vi "Find Tests.vi"(8 "error in (no error)":errorcluster, 10 "Project Refnum":refnum<vi>, 11 "LVUnit Test Discoverer in":refnum<class "LVUnit Test Discoverer.lvclass">) -> (0 "error out":errorcluster, 2 "Test Cases":refnum<class "Test Case.lvclass">[](array[class]), 3 "LVUnit Test Discoverer out":refnum<class "LVUnit Test Discoverer.lvclass">)   [LabVIEW 2017, in "LVUnit Test Discoverer.lvclass"]
doc: "Finds the tests available from the specified project refnum."
uses:
  LVUnit Test Discoverer.lvclass
  Test Case/Test Case.lvclass
  LVUnit Test Case/LVUnit Test Case.lvclass
  C:/Users/pasca/source/repos/lvunit/Test Case/Test Case.lvclass
  LVUnit Test Case/LVUnit Test Case.lvclass/LVUnit Test Case.ctl
  2d6a42ca-fa2d-47c0-93bd-f8bf5f61b6df.vi
  LVUnit Test Case/Set JSON Data.vi
  <vilib>/JDP Science/JSONtext/JSON text to Variant.vi
  <vilib>/JDP Science/JSONtext/LVClass Serializer/JSONtext LVClass Serializer.lvclass
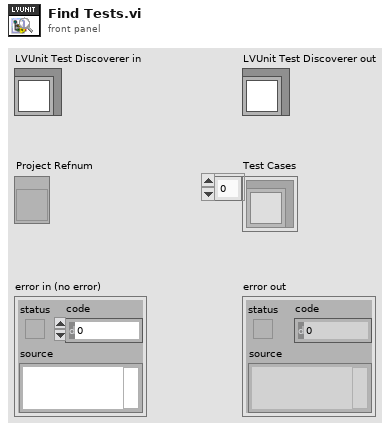
[diagram p1: front panel]
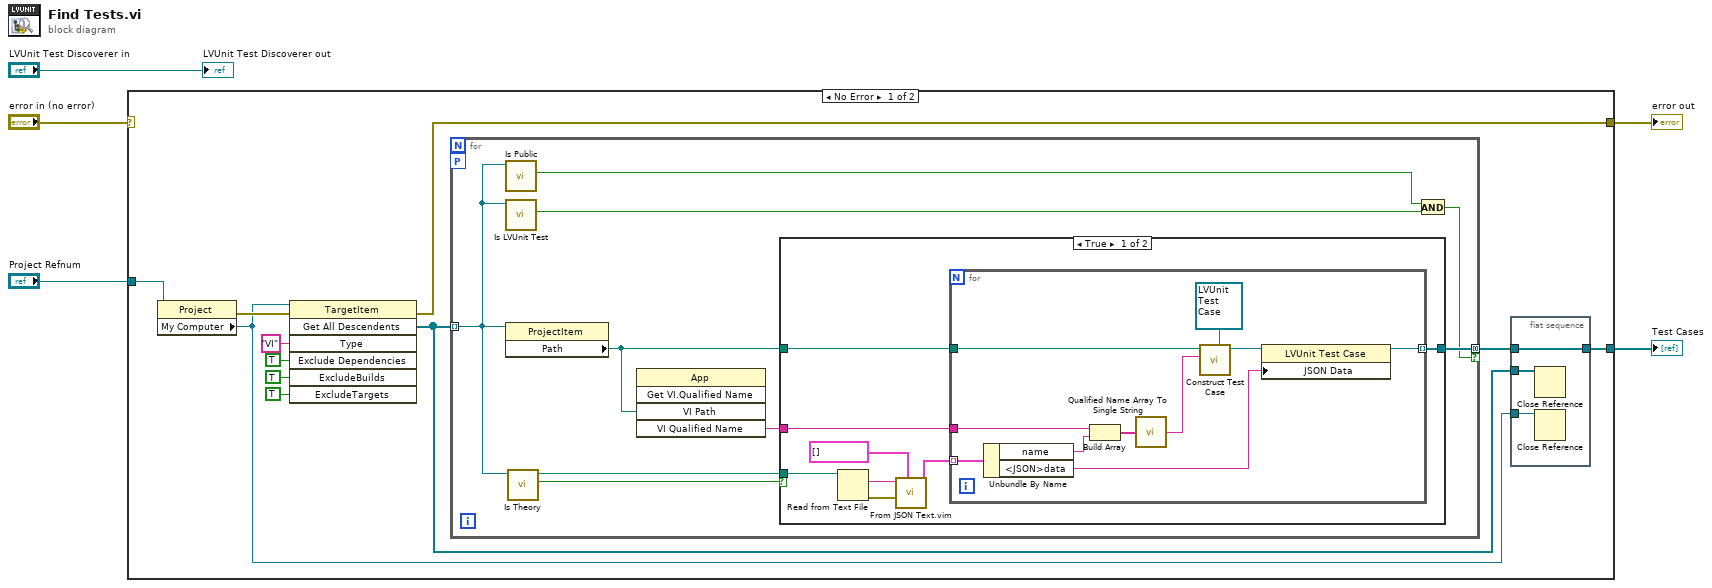
[diagram p0: block diagram]
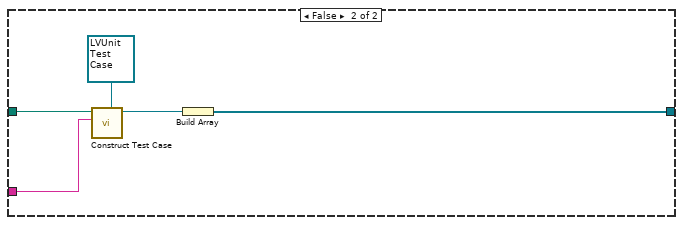
[diagram p2: hidden frame]
diagram:
  n1 = case shown="No Error" "error in (no error)" {
    selector: "error in (no error)" -> [_ w52]
    tunnel: "Project Refnum" -> [w16 _]
    tunnel: [w9 _] -> w3
    tunnel: [w12 w52] -> w2
    frame No Error {
      n2 = property class="Project"(reference=w16) -> (error out=w13:errorcluster, "My Computer"=w6:refnum<vi>)  [unwired: 1 in, 1 out]
      n3 = invoke class="TargetItem" method="Get All Descendents"(reference=w6, error in=w13, "Type"="VI", "Exclude Dependencies"=TRUE ("ExcludeDependencies"), "ExcludeBuilds"=TRUE, "ExcludeTargets"=TRUE) -> (error out=w12:errorcluster, "All Descendents"=w7:refnum<vi>[])  [unwired: 1 in, 5 out]
      n4 = for {
        tunnel: w7 -> [w25] mode=indexing
        tunnel: [w28] -> w8 mode=concatenating if=w22
        workers-P: _ -> [_]
        n5 = call "Is Public.vi"("ProjectItem Refnum"=w25) -> ("Is Public"=w23:bool)  [unwired: 10 in]
        n6 = call "Is LVUnit Test.vi"("ProjectItem Refnum"=w25) -> ("Is LVUnit Test"=w24:bool)  [unwired: 10 in]
        n7 = property class="ProjectItem"(reference=w25) -> ("Path"=w21:path)  [unwired: 1 in, 2 out]
        n8 = call "Is Theory.vi"("ProjectItem Refnum"=w25) -> ("Is Theory"=w26:bool, "Json File"=w27:path)  [unwired: 9 in]
        n9 = invoke class="App" method="Get VI.Qualified Name"("VI Path"=w21) -> ("VI Qualified Name"=w20:string)  [unwired: 4 in, 4 out]
        n10 = case shown="True" w26 {
          tunnel: [w36 w49] -> w28
          tunnel: w21 -> [w35 w50]
          tunnel: w27 -> [w30 _]
          tunnel: w20 -> [w34 w48]
          frame True {
            n11 = Read from Text File(file (use dialog)=w30) -> (text=w33:string, error out=w32:errorcluster)  [unwired: 3 in, 2 out]
            n12 = call "From JSON Text.vim"("Data Type and Default Value"=cluster{"name":string, "<JSON>data":string}[] [], "error in (no error)"=w32, "JSON"=w33) -> ("Data out"=w29:cluster{"name":string, "<JSON>data":string}[])  [unwired: 7 in, 1 out]
            n13 = for {
              tunnel: [w40] -> w36 mode=indexing
              tunnel: w35 -> [w45]
              tunnel: w34 -> [w44]
              tunnel: w29 -> [w39] mode=indexing
              n14 = Unbundle By Name(w39) -> ("name"=w38:string, "<JSON>data"=w37:string)
              n15 = Build Array(w44, w38) -> (w43:string[])
              n16 = call <vilib>:"Qualified Name Array To Single String.vi"("Fully Qualified Array"=w43) -> ("Fully Qualified String"=w42:string)
              n17 = call "Construct Test Case.vi"("Test Case in"=refnum<class "LVUnit Test Case.lvclass"> refnum ("LVUnit Test Case.lvclass"), "Qualified Name"=w42, "Path"=w45) -> ("Test Case out"=w46:refnum<class "LVUnit Test Case.lvclass">)  [unwired: 7 in, 1 out]
              n18 = property class="LVUnit Test Case"(reference=w46, "JSON Data"=w37) -> (reference out=w40:refnum<class "LVUnit Test Case.lvclass">)  [unwired: 1 in, 1 out]
            }
          }
          frame False {
            n19 = call "Construct Test Case.vi"("Test Case in"=refnum<class "LVUnit Test Case.lvclass"> refnum ("LVUnit Test Case.lvclass"), "Qualified Name"=w48, "Path"=w50) -> ("Test Case out"=w51:refnum<class "LVUnit Test Case.lvclass">)  [unwired: 7 in, 1 out]
            n20 = Build Array(w51) -> (w49:refnum<class "LVUnit Test Case.lvclass">[])
          }
        }
        n21 = And(x=w23, y=w24) -> (x .and. y?=w22:bool)
      }
      n22 = flat-sequence {
        tunnel: [w19] -> w9
        tunnel: w8 -> [w19]
        tunnel: w7 -> [w18]
        tunnel: w6 -> [w17]
        frame #0 {
          n23 = Close Reference(reference=w18) -> ()  [unwired: 1 in, 1 out]
          n24 = Close Reference(reference=w17) -> ()  [unwired: 1 in, 1 out]
        }
      }
    }
    frame Error {
    }
  }
  "error out" <- w2
  "Test Cases" <- w3
  "LVUnit Test Discoverer out" <- "LVUnit Test Discoverer in"
